vi "PicoScope2000ExampleStreaming.vi"() -> ()   [LabVIEW 2010]
doc: "This example demonstrates how to use the PicoScope Labview library to stream data from a PicoScope 2000 Series Device"
uses:
  PicoScope2000Lib/PicoScope2000AnalogChannelSettings.ctl
panel:
  out "overflow":i16 format="%02b"
  out "Unit Info":T1
  out "Channels App Buffer":cluster{i32, dbl, "Channel B Buffer":i16[]}[](graph)
  in  "AutoStop App Buffer":bool
  in  "Channel A Settings":T2={"Enabled"=TRUE, "Coupling"=1, "Range"=6} {"Range" items=["20 mV"=1, "50 mV"=2, "100 mV"=3, "200 mV"=4, "500 mV"=5, "1 V"=6, "2 V"=7, "5 V"=8, "10 V"=9, "20 V"=10]; "Coupling" items=["AC", "DC"]}
  in  "Channel B Settings":T2={"Enabled"=TRUE, "Coupling"=1, "Range"=6} {"Range" items=["20 mV"=1, "50 mV"=2, "100 mV"=3, "200 mV"=4, "500 mV"=5, "1 V"=6, "2 V"=7, "5 V"=8, "10 V"=9, "20 V"=10]; "Coupling" items=["AC", "DC"]}
  in  "Trigger Settings":T3={"Trigger Enabled"=FALSE, "Trigger Source"=enum."Channel A", "Trigger Threshold (V)"=0.0, "Trigger Direction"=0, "Trigger Delay (%)"=-50, "Auto Trigger Time (ms)"=1000} {"Trigger Direction" items=["Rising", "Falling"]; "Trigger Threshold (V)" format="%.3f"}
  out "Application Buffer Full":bool
  in  "Acquisition Settings":T4={"Auto Stop"=FALSE, "Desired Sample Interval"=2, "Max Samples"=333000, "Num Samples per Aggregate"=1, "Overview Buffer Size"=1000000, "Time Units"=3, "Application Buffer Size"=0} {"Time Units" items=["Nanoseconds (ns)"=2, "Microseconds (us)"=3, "Milliseconds (ms)"=4, "Seconds (s)"=5]; "Overview Buffer Size" format="%#.5p"; "Max Samples" format="%#.5p"}
  out "Analog Channels":T5(graph)
  out "Raw Sample Interval (sec)":dbl format="%#.5p"
  out "Chunk time":u32
  out "Elapsed time":dbl
  in  "Data file":path=path "PicoScope2000aExampleStreaming ChA Data"
  out "Queue depth ChA":i32(graph)
  out "queue depth":i32
  in  "Buffer and Transfer Settings":T6={"startIndex"=0, "Samples"=1500000, "Down Sample Ratio"=1, "Down-Sample Mode"=0} {"Down-Sample Mode" items=["None"=0, "Aggregate"=1, "Decimate"=2, "Average"=4]; "Down Sample Ratio" step=1; "Samples" format="%#_5p"}
  out "TriggeredAt (In Buffer)":u32 format="%#.6p"
  out "TriggeredAt (Total samples)":u32 format="%#.6p"
  out "Triggered":bool
  out "DownSample Interval (sec)":dbl format="%#.5p"
  out "Total Samples":u32 format="%#.6p"
  out "Auto Stopped":bool
  out "Number of Samples per Capture":u32 format="%#.6p"
  in  "Apply  Settings":bool
  in  "stop":bool
  # "Max. Recommended Settings\nSettings for 1 channels\nSample Interval 1 us\n\nSettings for 2 channels\nSample Interval 2 us\n\nRecommended Settings-\nMax. Samples 333k\nOverview Buffer 1M\n\nBuffer and Transfer Settings-\nSamples- 1.5M (as min.)\n(Buffer = x1.5 (min) Overview buffer)"
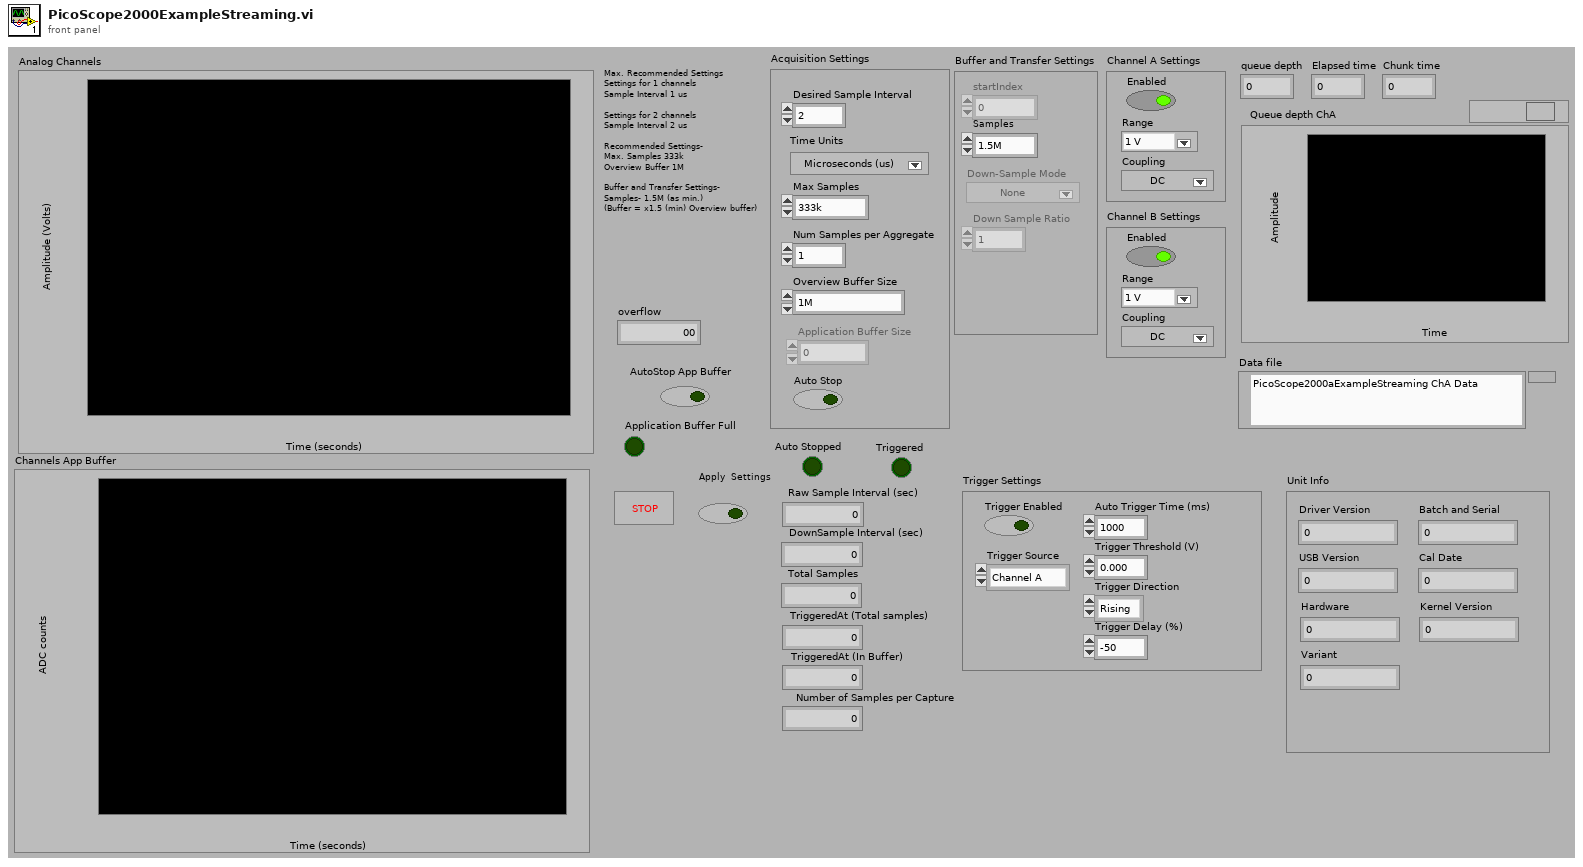
[diagram p1: front panel]
types:
  T1 = cluster{"Driver Version":string, "USB Version":string, "Hardware":string, "Variant":string, "Batch and Serial":string, "Cal Date":string, "Kernel Version":string}
  T2 = typedef "PicoScope2000AnalogChannelSettings.ctl" = cluster{"Enabled":bool, "Coupling":i16, "Range":u16}
  T3 = cluster{"Trigger Enabled":bool, "Trigger Source":enum16{"Channel A", "Channel B", "Channel C", "Channel D", "Ext."}, "Trigger Threshold (V)":dbl, "Trigger Direction":i16, "Trigger Delay (%)":i16, "Auto Trigger Time (ms)":i16}
  T4 = cluster{"Auto Stop":bool, "Desired Sample Interval":u32, "Max Samples":u32, "Num Samples per Aggregate":u32, "Overview Buffer Size":u32, "Time Units":u32, "Application Buffer Size":u32}
  T5 = cluster{i32, "DownSample Interval (sec)":dbl, "Data":dbl[]}[]
  T6 = cluster{"startIndex":u64, "Samples":u64, "Down Sample Ratio":u64, "Down-Sample Mode":u32}
  T7 = enum16{"open", "open or create", "create or replace", "create", "open (read-only)"}
  T8 = cluster{i32, "DownSample Interval (sec)":dbl, "Data":dbl[]}
  T9 = cluster{"Channel A Buffer":i16[], "Channel B Buffer":i16[], "Channel C Buffer":i16[], "Channel D Buffer":i16[], "Channel E Buffer":i16[], "Channel F Buffer":i16[], "Channel G Buffer":i16[], "Channel H Buffer":i16[], "Port 0":i16[], "Port 1":i16[]}
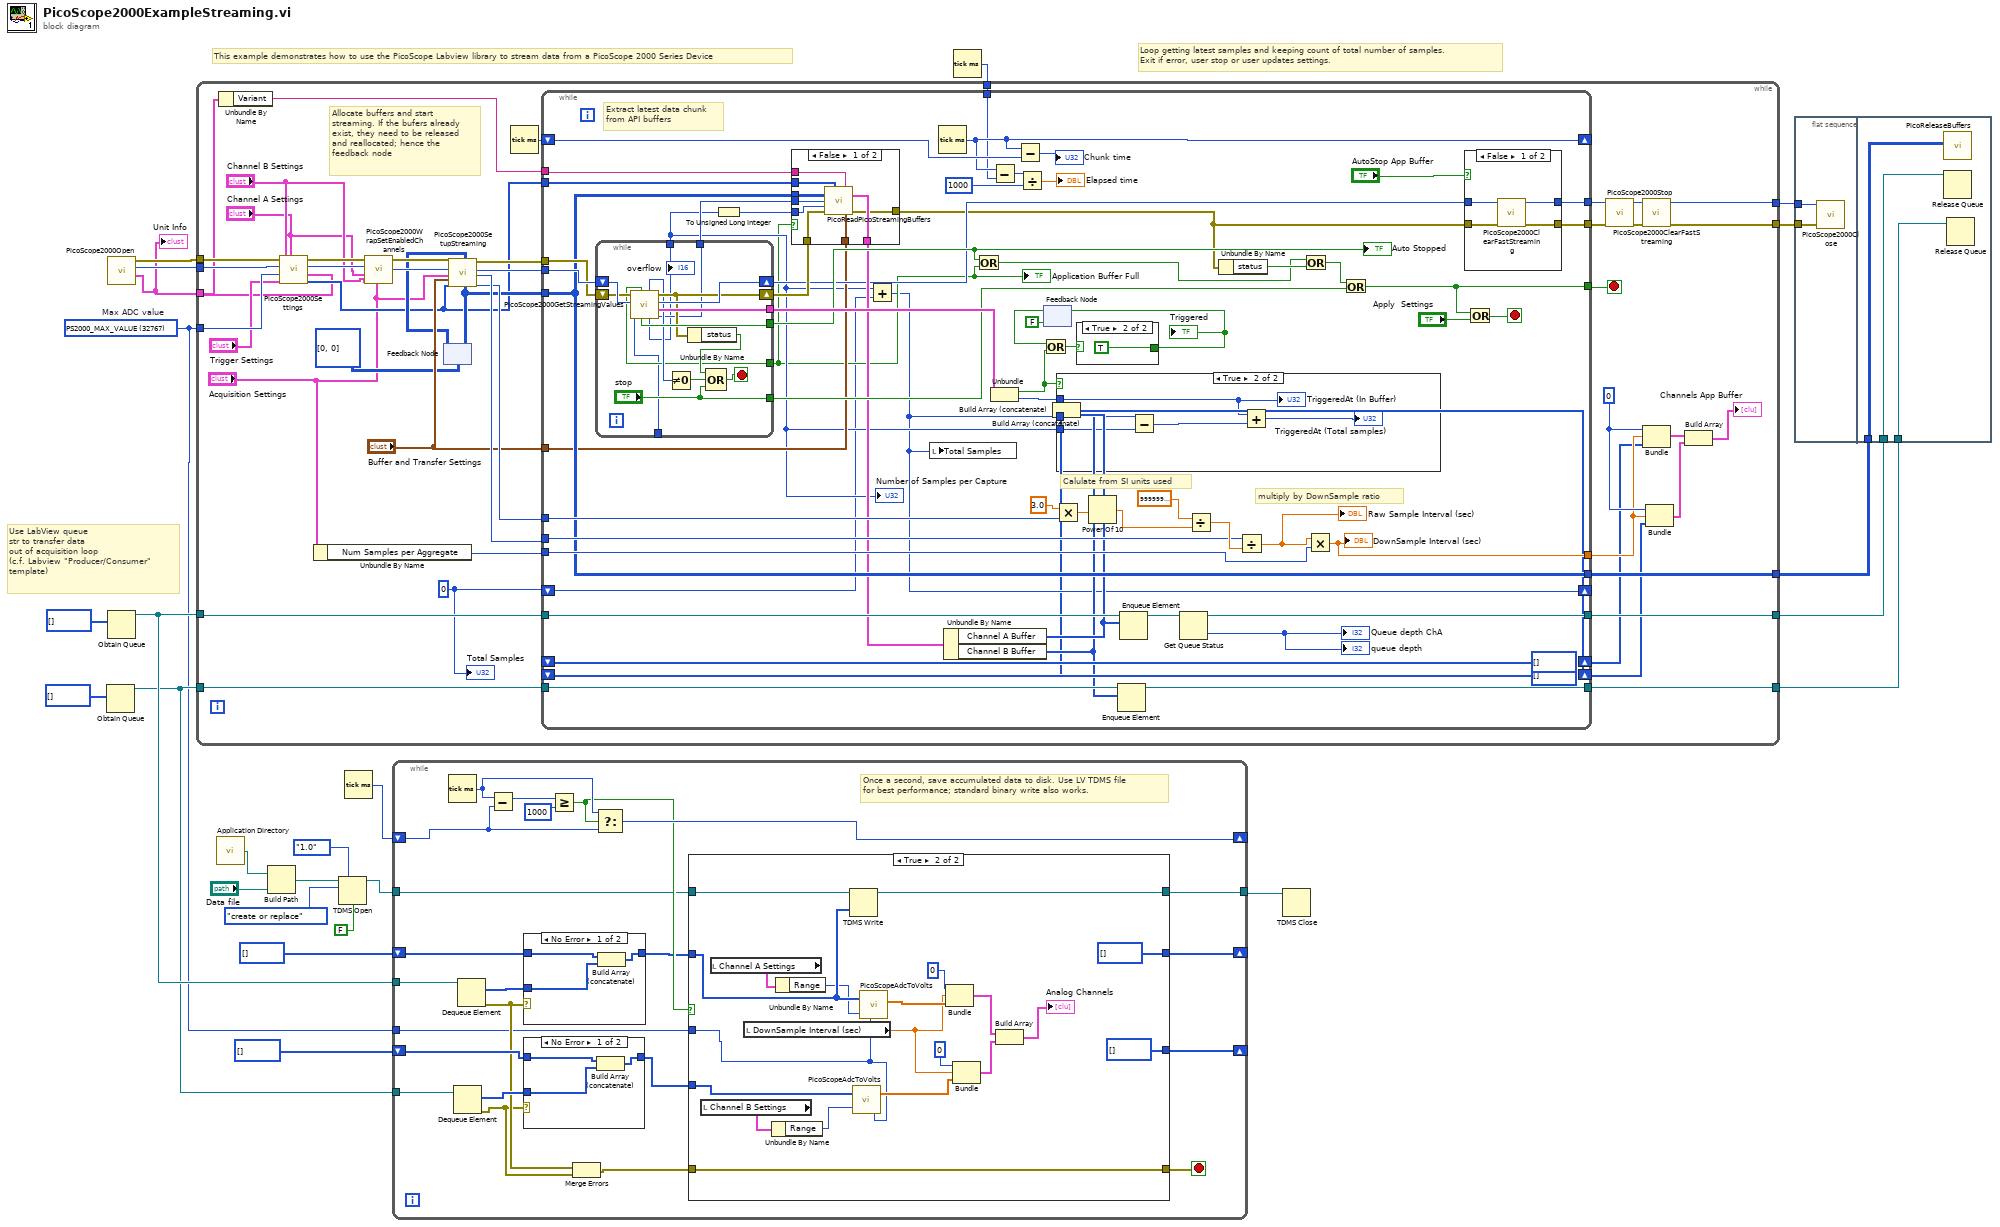
[diagram p0: block diagram]
diagram:
  w2 = i16 32767 items=["PS2000_MAX_VALUE"=32767]  # Max ADC value
  # "Loop getting latest samples and keeping count of total number of samples. \nExit if error, user stop or user updates settings."
  # "Use LabView queue\nstr to transfer data\nout of acquisition loop\n(c.f. Labview \"Producer/Consumer\"\ntemplate)"
  # "This example demonstrates how to use the PicoScope Labview library to stream data from a PicoScope 2000 Series Device"
  n1 = Obtain Queue(element data type=i16[] [] ("History Data")) -> (queue out=w3:refnum<queue>)  [unwired: 4 in, 2 out]
  n2 = call "PicoScope2000Open.vi"() -> ("Unit Info"=w1:T1, "handle"=w24:i16, "error out"=w25:errorcluster)  [unwired: 7 in]
  "Unit Info" <- w1
  n3 = Obtain Queue(element data type=i16[] [] ("History Data")) -> (queue out=w23:refnum<queue>)  [unwired: 4 in, 2 out]
  n4 = call <vilib>:"Application Directory.vi"() -> ("Application Directory"=w8:path)
  n5 = Build Path(base path=w8, name or relative path="Data file") -> (appended path=w9:path)
  n6 = TDMS Open(6:FALSE ("disable buffering? (T)"), 7:enum16{"1.0", "2.0"}."1.0" ("file format version (2.0)"), 10:T7."create or replace" ("operation (0:open)"), 11:w9) -> (3:w16:refnum<k34>)  [unwired: 2 in, 1 out]
  n7 = Tick Count (ms)() -> (millisecond timer value=w18:u32)
  n8 = while {
    tunnel: w23 -> [w47]
    shift-right: [w38] -> _
    shift-left: i16[] [] ("History Data") -> [w46]
    shift-right: [w41] -> _
    shift-left: w18 -> [w42]
    tunnel: w16 -> [w37]
    tunnel: [w36] -> w15
    tunnel: w3 -> [w35]
    shift-right: [w31] -> _
    shift-left: i16[] [] ("History Data") -> [w34]
    tunnel: w2 -> [w26]
    stop <- w28 stop-if-true
    # "Once a second, save accumulated data to disk. Use LV TDMS file\nfor best performance; standard binary write also works."
    n9 = Tick Count (ms)() -> (millisecond timer value=w43:u32)
    n10 = Dequeue Element(queue=w35) -> (element=w33:i16[], error out=w29:errorcluster)  [unwired: 2 in, 2 out]
    n11 = Dequeue Element(queue=w47) -> (element=w48:i16[], error out=w30:errorcluster)  [unwired: 2 in, 2 out]
    n12 = Subtract(x=w43, y=w42) -> (x-y=w45:u32)
    n13 = case shown="No Error" w29 {
      tunnel: w34 -> [w51 w52]
      tunnel: [w50 w52] -> w32
      tunnel: w33 -> [w49 _]
      frame No Error {
        n14 = Build Array (concatenate)(w51, w49) -> (w50:i16[])
      }
      frame Error {
      }
    }
    n15 = case shown="No Error" w30 {
      tunnel: w46 -> [w79 w80]
      tunnel: [w78 w80] -> w39
      tunnel: w48 -> [w77 _]
      frame No Error {
        n16 = Build Array (concatenate)(w79, w77) -> (w78:i16[])
      }
      frame Error {
      }
    }
    n17 = Greater Or Equal?(x=w45, y=u32 1000) -> (x >= y?=w40:bool)
    n18 = Merge Errors(w30, w29) -> (w27:errorcluster)
    n19 = Select(t=w43, s=w40, f=w42) -> (s? t:f=w41:u32)
    n20 = case shown="True" w40 {
      tunnel: w39 -> [w56 w73]
      tunnel: [w56 i16[] [] ("History Data")] -> w38
      tunnel: w37 -> [w55 w75]
      tunnel: [w55 w74] -> w36
      tunnel: w32 -> [w54 w61]
      tunnel: [w54 i16[] [] ("History Data")] -> w31
      tunnel: [w53 w58] -> w28
      tunnel: w27 -> [w53 w58]
      tunnel: w26 -> [_ w57]
      frame False {
      }
      frame True {
        n21 = local read "Channel B Settings"() -> (w60:T2)
        n22 = local read "Channel A Settings"() -> (w69:T2)
        n23 = local read "DownSample Interval (sec)"() -> (w64:dbl)
        n24 = Unbundle By Name(w60) -> ("Range"=w62:u16)
        n25 = Unbundle By Name(w69) -> ("Range"=w72:u16)
        n26 = TDMS Write(0:w75, 9:w73) -> (4:w74:refnum<k34>)  [unwired: 4 in, 3 out]
        n27 = call "PicoScopeAdcToVolts.vi"("Max_adc"=w57, "Range Index"=w62, "Data"=w61) -> ("Data"=w63:dbl[])
        n28 = call "PicoScopeAdcToVolts.vi"("Max_adc"=w57, "Range Index"=w72, "Data"=w73) -> ("Data"=w70:dbl[])
        n29 = Bundle(0, "DownSample Interval (sec)"=w64, "Data"=w70) -> (w67:T8)  [unwired: 1 in]
        n30 = Bundle(0, "DownSample Interval (sec)"=w64, "Data"=w63) -> (w66:T8)  [unwired: 1 in]
        n31 = Build Array(w67, w66) -> (→"Analog Channels":T5)
      }
    }
  }
  n32 = Tick Count (ms)() -> (millisecond timer value=w22:u32)
  n33 = while {
    tunnel: [w83] -> w21
    tunnel: w25 -> [w125]
    tunnel: w24 -> [w126]
    tunnel: w1 -> [w102]
    tunnel: w2 -> [w107]
    tunnel: [w115] -> w19
    tunnel: w23 -> [w114]
    tunnel: [w113] -> w20
    tunnel: w22 -> [w110]
    tunnel: [w84] -> w7
    tunnel: w3 -> [w98]
    tunnel: [w97] -> w5
    stop <- w127 stop-if-true
    w96 = 0
    w87 = u32 0 ("Total Samples")
    # "Allocate buffers and start\nstreaming. If the bufers already\nexist, they need to be released\nand reallocated; hence the\nfeedback node"
    n34 = Unbundle By Name(w102) -> ("Variant"=w101:string)
    n35 = call "PicoScope2000Settings.vi"("Unit Info"=w102, "Channel B Settings"="Channel B Settings", "Channel A Settings"="Channel A Settings", "Trigger Settings"="Trigger Settings", "Max ADC value"=w107, "handle in"=w126, "error in"=w125) -> ("Enabled Array"=w106:i16[], "handle out"=w119:i16, "error out"=w120:errorcluster)
    n36 = Unbundle By Name("Acquisition Settings") -> ("Num Samples per Aggregate"=w89:u32)
    n37 = call "PicoScope2000WrapSetEnabledChannels.vi"("Acquisition Settings"="Acquisition Settings", "Channel B Settings"="Channel B Settings", "Channel A Settings"="Channel A Settings", "handle in"=w119, "error in (no error)"=w120) -> ("handle out"=w122:i16, "error out"=w121:errorcluster)  [unwired: 1 in]
    n38 = feedback #1(u64[][] [[0], [0]] ("Pointer array")) -> (w112:u64[][])
    n39 = call "PicoScope2000SetupStreaming.vi"("error in"=w121, "handle in"=w122, "Acquisition Settings"="Acquisition Settings", "Buffer and Transfer Settings"="Buffer and Transfer Settings", "enabled array"=w106, "Pointers In"=w112) -> ("Pointer array"=w109:u64[][], "error out"=w123:errorcluster, "handle out"=w124:i16, "Sample Interval"=w118:u32, "sampleIntervalTimeUnits"=w117:u32)  [unwired: 9 in]
    n40 = feedback-in #1(w109) -> ()
    n41 = Tick Count (ms)() -> (millisecond timer value=w111:u32)
    n42 = while {
      tunnel: [w147] -> w100
      tunnel: [w189] -> w127
      tunnel: w124 -> [w170]
      tunnel: w123 -> [w169]
      tunnel: w118 -> [w172]
      tunnel: w117 -> [w179]
      tunnel: [w146] -> w99
      tunnel: w89 -> [w171]
      tunnel: "Buffer and Transfer Settings" -> [w144]
      tunnel: w106 -> [w167]
      tunnel: [w165] -> w115
      tunnel: w114 -> [w163]
      tunnel: w109 -> [w162]
      tunnel: [w162] -> w113
      shift-right: [w157] -> _
      shift-left: w111 -> [w158]
      tunnel: w110 -> [w156]
      tunnel: w101 -> [w154]
      tunnel: w98 -> [w137]
      tunnel: [w136] -> w97
      tunnel: [w135] -> w92
      shift-right: [w133] -> _
      shift-left: w87 -> [w132]
      shift-right: [w130] -> w91
      shift-left: i16[] [] ("Channel A Buffer") -> [w131]
      shift-right: [w128] -> w90
      shift-left: i16[] [] ("Channel B Buffer") -> [w129]
      stop <- w188 stop-if-true
      # "Extract latest data chunk\nfrom API buffers"
      # "Calulate from SI units used"
      # "multiply by DownSample ratio"
      n43 = while {
        tunnel: [w221] -> w187
        tunnel: [w220] -> w151
        tunnel: [w209] -> w142
        tunnel: [w208] -> w141
        shift-right: [w217] -> w148
        shift-left: w170 -> [w219]
        shift-right: [w216] -> w168
        shift-left: w169 -> [w218]
        tunnel: ["stop"] -> w152
        tunnel: [w210] -> w140
        tunnel: [w207] -> _
        stop <- w212 stop-if-true
        n44 = call "PicoScope2000GetStreamingValues.vi"("handle in"=w219, "error in"=w218) -> ("App Buffer startIndex"=w209:u32, "Trigger"=w221:cluster{bool, "triggeredAt  Index (Total)":u32}, "handle out"=w217:i16, "error out"=w216:errorcluster, "Number of Samples"=w208:u32, "ready"=w215:i16, "Auto Stopped"=w220:bool, "Application Buffer Full"=w210:bool, "overflow"=w207:i16)  [unwired: 1 out]
        n45 = Not Equal To 0?(x=w215) -> (x != 0?=w213:bool)
        n46 = Unbundle By Name(w216) -> ("status"=w214:bool)
        n47 = Compound Arithmetic op=OR(w214, w213, "stop") -> (w212:bool)
      }
      "Number of Samples per Capture" <- w141
      "Auto Stopped" <- w151
      "Application Buffer Full" <- w140
      n48 = To Unsigned Long Integer(number=w141) -> (unsigned 32bit integer=w143:u32)
      n49 = case shown="False" w140 {
        tunnel: w168 -> [w205 w206]
        tunnel: w167 -> [w204 _]
        tunnel: w162 -> [w203 _]
        tunnel: w154 -> [w202 _]
        tunnel: [w201 _] -> w149
        tunnel: [w200 w206] -> w145
        tunnel: w144 -> [w199 _]
        tunnel: w143 -> [w198 _]
        tunnel: w142 -> [w197 _]
        frame False {
          n50 = call "PicoReadPicoStreamingBuffers.vi"("enabled array"=w204, "Buffer and Transfer Settings"=w199, "Variant"=w202, "Pointer array"=w203, "Offset Index"=w197, "Number of Samples"=w198, "error in (no error)"=w205) -> ("Buffers (Max or non-aggregated)"=w201:T9, "error out"=w200:errorcluster)  [unwired: 6 in, 1 out]
        }
        frame True {
        }
      }
      n51 = Add(x=w141, y=w132) -> (x+y=w133:u32)
      n52 = local write "Total Samples"(w133) -> ()
      n53 = Tick Count (ms)() -> (millisecond timer value=w157:u32)
      n54 = Unbundle By Name(w149) -> ("Channel A Buffer"=w139:i16[], "Channel B Buffer"=w134:i16[])
      n55 = Or(x=w151, y=w140) -> (x .or. y?=w150:bool)
      n56 = Subtract(x=w157, y=w156) -> (x-y=w161:u32)
      n57 = Unbundle(w187) -> (w174:bool, "triggeredAt  Index (Total)"=w173:u32)
      n58 = Subtract(x=w157, y=w158) -> (x-y=→"Chunk time":u32)
      n59 = Divide(x=w161, y=u32 1000) -> (x/y=→"Elapsed time":dbl)
      n60 = feedback #2(FALSE) -> (w184:bool)
      n61 = Or(x=w184, y=w174) -> (x .or. y?=w176:bool)
      n62 = Build Array (concatenate)(w129, w134) -> (w128:i16[])
      n63 = Build Array (concatenate)(w131, w139) -> (w130:i16[])
      n64 = Multiply(x=3.0, y=w179) -> (x*y=w177:dbl)
      n65 = case shown="True" w174 {
        tunnel: w141 -> [_ w222]
        tunnel: w133 -> [_ w226]
        tunnel: w173 -> [_ w224]
        frame False {
        }
        frame True {
          n66 = Subtract(x=w226, y=w222) -> (x-y=w225:u32)
          n67 = Add(x=w224, y=w225) -> (x+y=→"TriggeredAt (Total samples)":u32)
          "TriggeredAt (In Buffer)" <- w224
        }
      }
      n68 = case shown="True" w176 {
        selector: w176 -> [w227 _]
        tunnel: [w227 TRUE] -> w175
        frame False {
        }
        frame True {
        }
      }
      "Triggered" <- w175
      n69 = feedback-in #2(w175) -> ()
      n70 = Power Of 10(x=w177) -> (10^x=w178:dbl)
      n71 = Enqueue Element(queue=w137, element=w134) -> (queue out=w136:refnum<queue>)  [unwired: 2 in, 2 out]
      n72 = Enqueue Element(queue=w163, element=w139) -> (queue out=w164:refnum<queue>)  [unwired: 2 in, 2 out]
      n73 = Get Queue Status(queue=w164) -> (queue out=w165:refnum<queue>, # elements in queue=→"queue depth" →"Queue depth ChA":i32)  [unwired: 2 in, 6 out]
      n74 = Divide(x=sgl 1000000000000000.0 ("y"), y=w178) -> (x/y=w180:dbl)
      n75 = Unbundle By Name(w145) -> ("status"=w186:bool)
      n76 = Divide(x=w172, y=w180) -> (x/y=w153:dbl)
      "Raw Sample Interval (sec)" <- w153
      n77 = Or(x=w150, y=w186) -> (x .or. y?=w185:bool)
      n78 = Multiply(x=w153, y=w171) -> (x*y=w135:dbl)
      "DownSample Interval (sec)" <- w135
      n79 = Or(x=w185, y=w152) -> (x .or. y?=w189:bool)
      n80 = case shown="False" "AutoStop App Buffer" {
        tunnel: w148 -> [w194 w195]
        tunnel: [w191 w195] -> w147
        tunnel: [w192 w196] -> w146
        tunnel: w145 -> [w193 w196]
        frame False {
          n81 = call "PicoScope2000ClearFastStreaming.vi"("error in"=w193, "handle"=w194) -> ("error out"=w192:errorcluster, "handle out"=w191:i16)  [unwired: 4 in]
        }
        frame True {
        }
      }
      n82 = Or(x=w189, y="Apply  Settings") -> (x .or. y?=w188:bool)
    }
    n83 = call "PicoScope2000Stop.vi"("error in (no error)"=w99, "handle in"=w100) -> ("error out"=w86:errorcluster, "handle out"=w85:i16)  [unwired: 8 in]
    n84 = call "PicoScope2000ClearFastStreaming.vi"("error in"=w86, "handle"=w85) -> ("error out"=w84:errorcluster, "handle out"=w83:i16)  [unwired: 4 in]
    n85 = Bundle(w96, w92, "Channel A Buffer"=w91) -> (w95:cluster{i32, dbl, "Channel A Buffer":i16[]})  [unwired: 1 in]
    n86 = Bundle(w96, w92, "Channel B Buffer"=w90) -> (w94:cluster{i32, dbl, "Channel B Buffer":i16[]})  [unwired: 1 in]
    n87 = Build Array(w95, w94) -> (→"Channels App Buffer":cluster{i32, dbl, "Channel B Buffer":i16[]}[])
    "Total Samples" <- w87
  }
  n88 = TDMS Close(11:w15) -> ()  [unwired: 1 in, 2 out]
  n89 = flat-sequence {
    tunnel: w21 -> [w230]
    tunnel: w7 -> [w229]
    tunnel: w20 -> [w233]
    tunnel: w19 -> [w232]
    tunnel: w5 -> [w231]
    frame #0 {
      n90 = call "PicoScope2000Close.vi"("error in"=w229, "handle"=w230) -> ()  [unwired: 4 in, 2 out]
    }
    frame #1 {
      n91 = call "PicoReleaseBuffers.vi"("Pointer array"=w233) -> ()  [unwired: 10 in, 1 out]
      n92 = Release Queue(queue=w232) -> ()  [unwired: 2 in, 3 out]
      n93 = Release Queue(queue=w231) -> ()  [unwired: 2 in, 3 out]
    }
  }
